vi "movetest.vi"() -> ()   [LabVIEW 2019]
panel:
  out "error out":errorcluster
  in  "error in (no error)":errorcluster
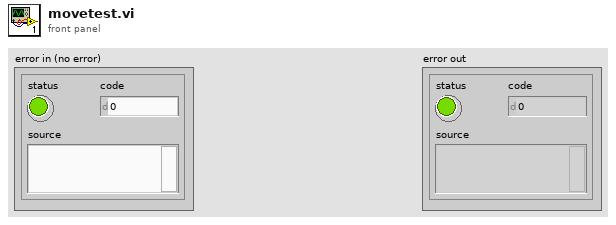
[diagram p1: front panel]
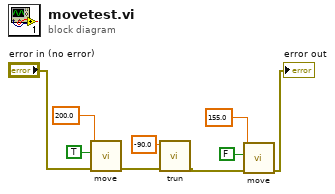
[diagram p0: block diagram]
diagram:
  n1 = call "move.vi"("error in (no error)"="error in (no error)", "タは"=TRUE, "移動距離"=200.0) -> ("error out"=w4:errorcluster)  [unwired: 8 in]
  n2 = call "trun.vi"("error in (no error)"=w4, "旋轉"=-90.0) -> ("error out"=w9:errorcluster)  [unwired: 9 in]
  n3 = call "move.vi"("error in (no error)"=w9, "タは"=FALSE, "移動距離"=155.0) -> ("error out"=→"error out":errorcluster)  [unwired: 8 in]
